vi "get_chirp_point_nowindow__e18cf5ad44.vi"(0 "relative seconds":dbl, 1 "omega2":dbl=1.0 format="%0.2f", 2 "Duration":dbl, 4 "window":bool, 5 "voltage to displacement constant":dbl, 7 "Initial position in voltage":dbl, 9 "amplitude":dbl=1.0 format="%0.2f", 11 "omega1":dbl=1.0 format="%0.2f", 12 "r":dbl, 13 "p":dbl) -> (3 "set point":dbl, 14 "Elapsedf time (s)":dbl)   [LabVIEW 2023]
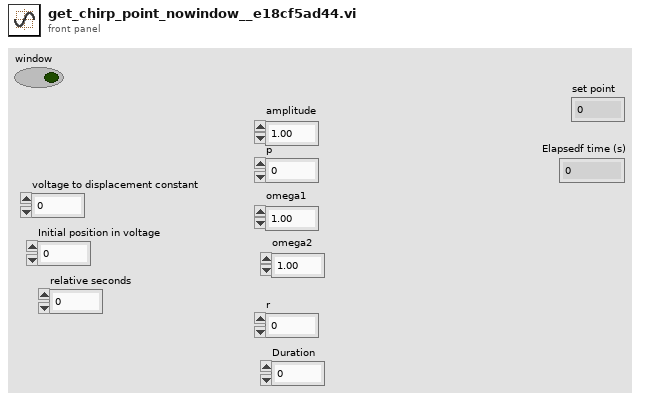
[diagram p1: front panel]
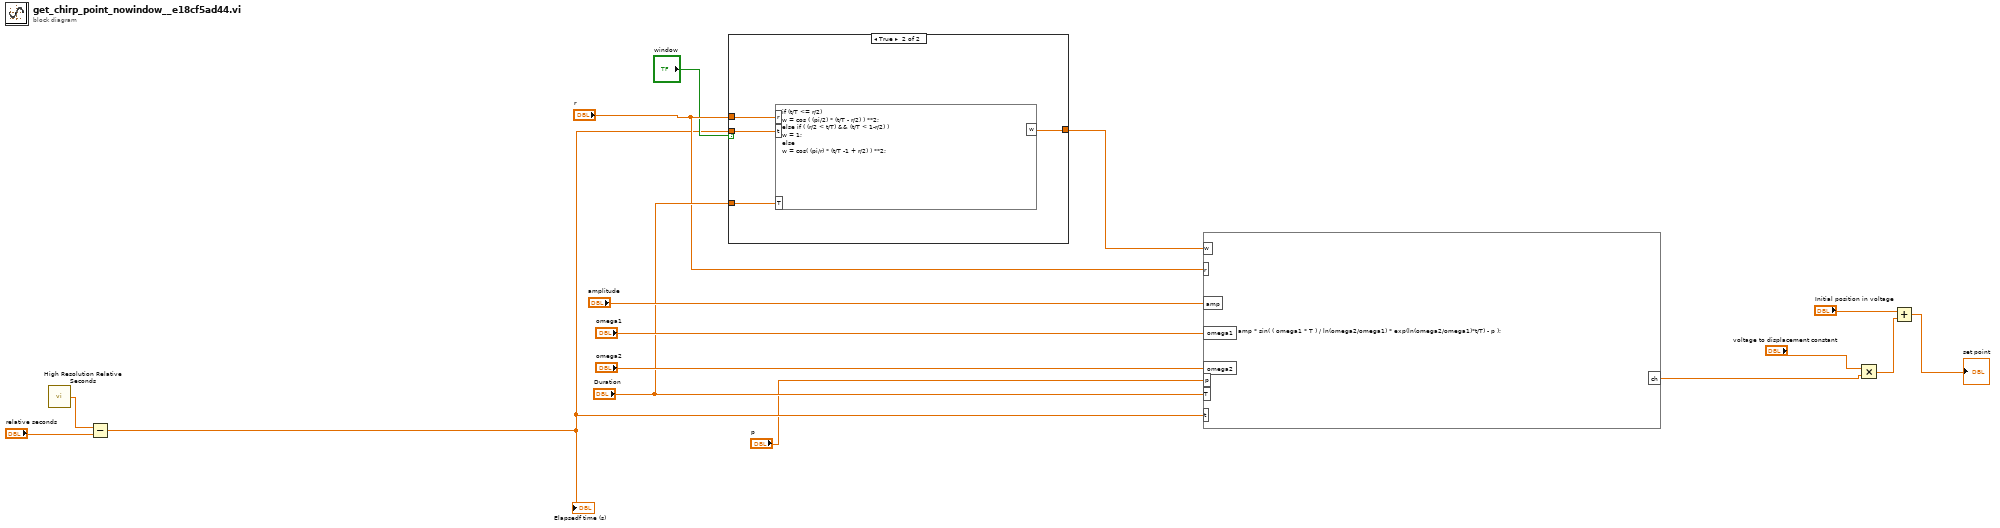
[diagram p0: block diagram]
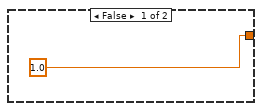
[diagram p2: hidden frame]
diagram:
  n1 = call <vilib>:"High Resolution Relative Seconds.vi"() -> ("relative seconds"=w15:dbl)
  n2 = Subtract(x=w15, y="relative seconds") -> (x-y=w2:dbl)
  "Elapsedf time (s)" <- w2
  n3 = case shown="True" "window" {
    tunnel: "Duration" -> [_ w21]
    tunnel: "r" -> [_ w20]
    tunnel: [1.0 w19] -> w7
    tunnel: w2 -> [_ w18]
    frame False {
    }
    frame True {
      n4 = formula code="if (t/T <= r/2) \nw = cos ( (pi/2) * (t/T - r/2) ) **2;\nelse if ( (r/2 < t/T) && (t/T < 1-r/2) )\nw = 1;\nelse\nw = cos( (pi/r) * (t/T -1 + r/2) ) **2;"("r"=w20, "t"=w18, "T"=w21) -> ("w"=w19:dbl)
    }
  }
  n5 = formula code="ch = w * amp * sin( ( omega1 * T ) / ln(omega2/omega1) * exp(ln(omega2/omega1)*t/T) - p );"("amp"="amplitude", "omega1"="omega1", "omega2"="omega2", "T"="Duration", "t"=w2, "r"="r", "w"=w7, "p"="p") -> ("ch"=w5:dbl)
  n6 = Multiply(x="voltage to displacement constant", y=w5) -> (x*y=w3:dbl)
  n7 = Add(x="Initial position in voltage", y=w3) -> (x+y=→"set point":dbl)
